vi "Get All Tags.vi"(8 "error in (no error)":errorcluster) -> (0 "error out":errorcluster, 2 "Tag Refs":refnum<data-value>[](array[refnum]))   [LabVIEW 2020, in "Tag Engine Core.lvlib" / "Tag Core.lvclass"]
doc: "_SubVI_"
uses:
  Tag Core.lvclass
  Tag/Tag.lvclass
  Tag Core.lvclass/Tag Core.ctl
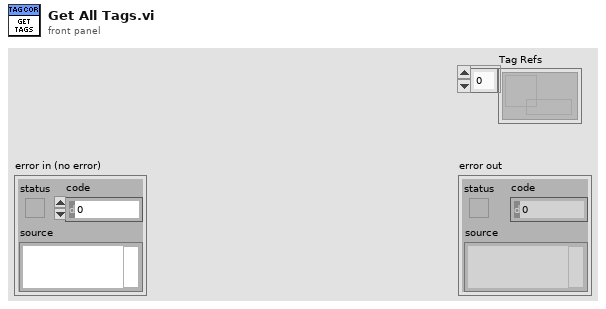
[diagram p1: front panel]
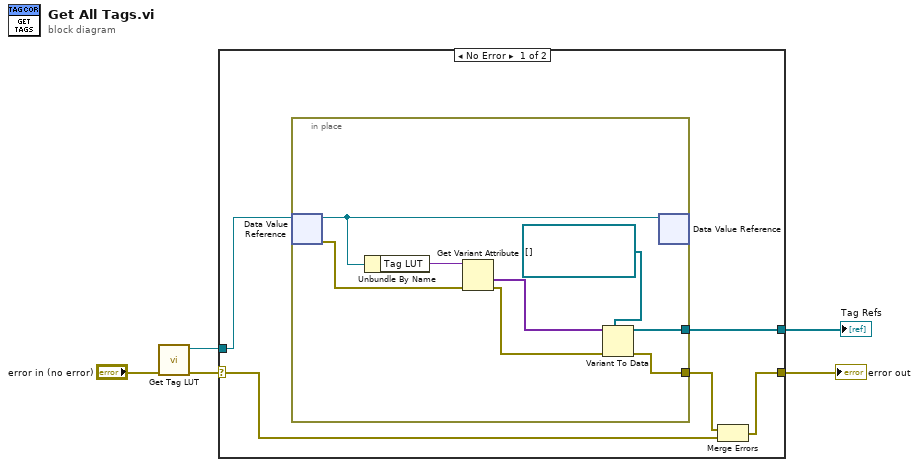
[diagram p0: block diagram]
diagram:
  n1 = call "Get Tag LUT.vi"("error in (no error)"="error in (no error)") -> ("error out"=w2:errorcluster, "Tag LUT Out"=w1:refnum<data-value>)  [unwired: 9 in]
  n2 = case shown="No Error" w2 {
    selector: w2 -> [w9 w19]
    tunnel: [w7 w19] -> w5
    tunnel: w1 -> [w10 _]
    tunnel: [w6 _] -> w4
    frame No Error {
      n3 = in-place {
        in-place-border: [w15] -> w6
        in-place-border: [w12] -> w8
        n4 = in-place-dvr #1(w10) -> (w18:refnum<class "Tag Core.lvclass">, w14:errorcluster)
        n5 = Unbundle By Name(w18) -> ("Tag LUT"=w17:variant)
        n6 = Get Variant Attribute(Variant=w17, error in=w14) -> (values=w16:variant[], error out=w13:errorcluster)  [unwired: 2 in, 2 out]
        n7 = Variant To Data(error in=w13, type=refnum<data-value>[] [] ("CVT Item in"), Variant=w16) -> (data=w15:refnum<data-value>[], error out=w12:errorcluster)
        n8 = in-place-dvr #1(w18) -> ()  [unwired: 2 out]
      }
      n9 = Merge Errors(w8, w9) -> (w7:errorcluster)
    }
    frame Error {
    }
  }
  "error out" <- w5
  "Tag Refs" <- w4
